vi "Mandelbrot_Top.vi"() -> ()   [LabVIEW 2020]
doc: "This benchmark is designed to demonstrate execution performance improvement when executing FFT and IFFT operations on a GPU."
uses:
  <vilib>/Analysis/1siggen.llb/Ramp Pattern by Delta.vi
  <vilib>/Utility/file.llb/Read Delimited Spreadsheet (DBL).vi
  <vilib>/Ngene/CuLab - GPU Accelerated Toolkit/Toolkit/CuLab.lvlib
  <vilib>/Analysis/NI_AALBase.lvlib
panel:
  out "CuLab Mean Performance Gain":dbl[](array[numeric])=[1.0, 22.05888198839261, 2.294988144455706] format="%#.2g"
  out "Releative Exec Time vs CuLab":cluster{i32[], "all rows":dbl[]}[](graph)=[{[100, 200, 300, 400, 500, 600, 700, 800, 900, 1000], "all rows"=[1.0, 1.0, 1.0, 1.0, 1.0, 1.0, 1.0, 1.0, 1.0, 1.0]}, {[100, 200, 300, 400, 500, 600, 700, 800, 900, 1000], "all rows"=[0.8045912431423006, 2.8737294623342633, 6.2281949138049875, 11.291126277991692, 18.815012396949246, 27.10316550048527, 34.90172708957351, 38.99811295548449, 39.49387679077455, 40.07928325338579]}, {[100, 200, 300, 400, 500, 600, 700, 800, 900, 1000], "all rows"=[2.9876362098895357, 2.6173252742418085, 2.4274383662643, 2.414197215437082, 2.5477456703897334, 2.477240832223878, 2.3481639475839504, 2.0064648536535485, 1.786744893645114, 1.336924181228108]}]
  in  "CuPy CSV":path=path "D:/Ngene/GitHub/culab_examples/Benchmarks/CuPy/results/GeForce_RTX_2080_Ti/Mandelbrot_CuPy.csv"
  out "Execution Time":cluster{i32[], "FFT mean Exec Time":dbl[]}[](graph)=[{[100, 200, 300, 400, 500, 600, 700, 800, 900, 1000], "FFT mean Exec Time"=[0.1258352000004379, 0.13859289999982138, 0.1453709000006711, 0.14599060000000463, 0.1388639000006151, 0.14194279999992432, 0.1489036999992095, 0.17667840000012802, 0.22171379999963392, 0.26985270000022865]}, {[100, 200, 300, 400, 500, 600, 700, 800, 900, 1000], "FFT mean Exec Time"=[0.10124589999941236, 0.398278499999833, 0.9053982999994332, 1.6483982999998261, 2.6127260000002934, 3.8470992000002298, 5.196996300000137, 6.8901241999992635, 8.756337499999972, 10.815502800000104]}, {[100, 200, 300, 400, 500, 600, 700, 800, 900, 1000], "FFT mean Exec Time"=[0.3759498, 0.36274270000000003, 0.3528789, 0.35245010000000004, 0.35378990000000005, 0.3516265, 0.3496503, 0.354499, 0.396146, 0.3607726]}]
  in  "Size Delta":i32=100
  out "GPU Model":string="NVIDIA GeForce RTX 2080 Ti"
  out "CPU Model":string="Intel(R) Core(TM) i7-8700K"
  in  "Max Iterations":i32=1000
  in  "Size Stop":i32=1000
  in  "Size Start":i32=100
  out "Dims H,W":i32[](array[numeric])=[100, 200, 300, 400, 500, 600, 700, 800, 900, 1000] format="%.2p"
  # "Mandelbrot Benchmark"
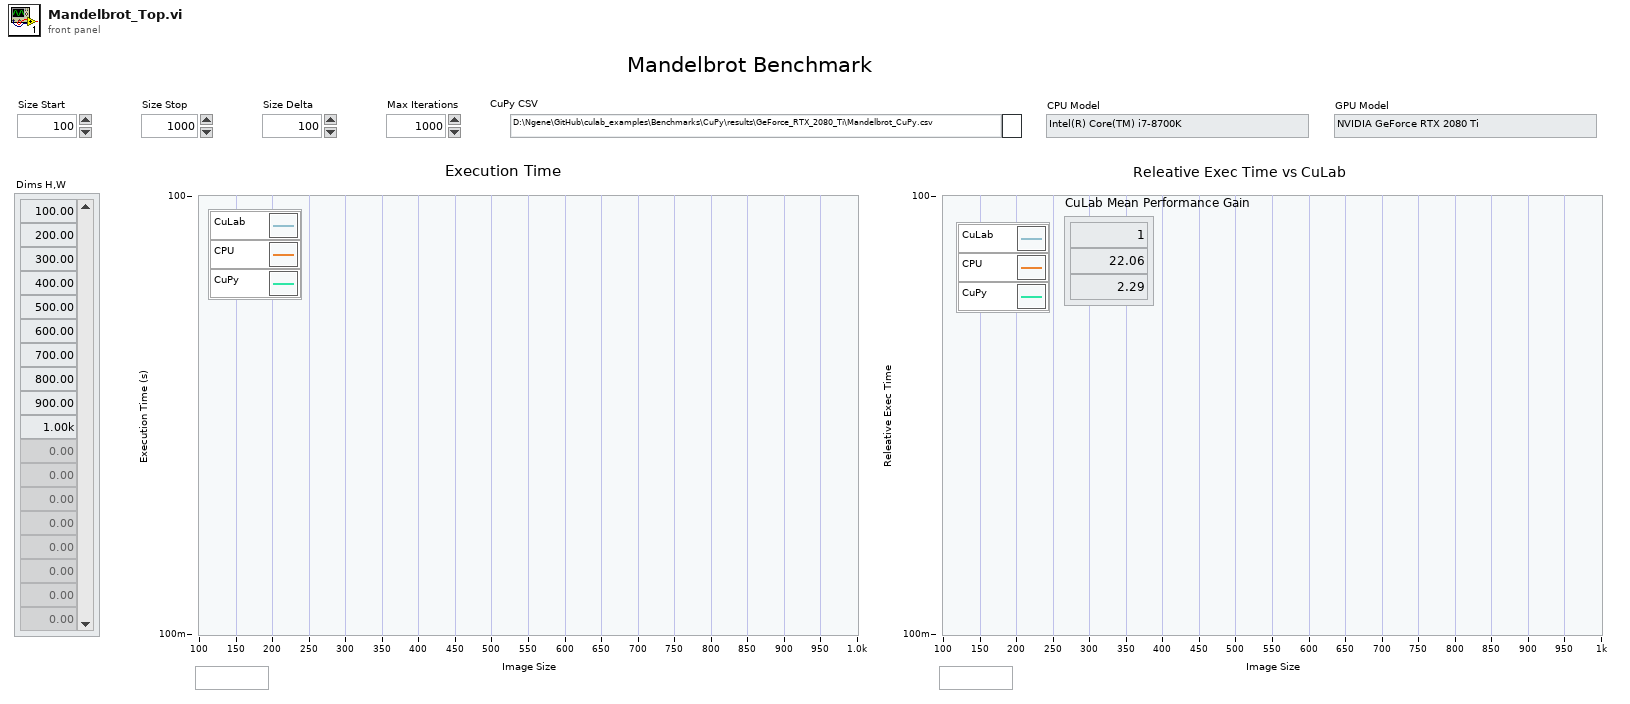
[diagram p1: front panel]
types:
  T1 = typedef "CuLab.lvlib/Properties.ctl" = cluster{"Device ID":i32, "Name":string}
  T2 = typedef "imagedata.ctl" = cluster{"image type":i32, "image depth":i32, "image":u8[], "mask":u8[], "colors":u32[], "Rectangle":cluster{"left":i16, "top":i16, "right":i16, "bottom":i16}}
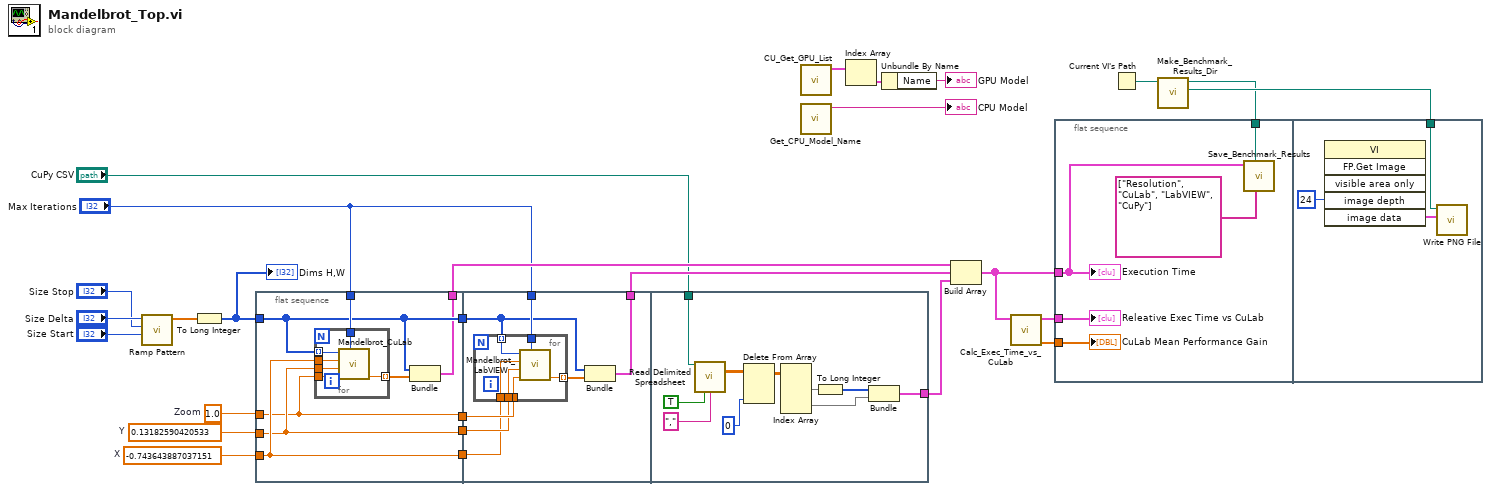
[diagram p0: block diagram]
diagram:
  w15 = 1.0  # Zoom
  w16 = 0.13182590420533  # Y
  w17 = -0.743643887037151  # X
  n1 = call-poly <vilib>:"Ramp Pattern.vi"("start"="Size Start", "end"="Size Stop", "delta"="Size Delta") -> ("Ramp Pattern"=w19:dbl[])  [unwired: 6 in, 2 out]
  n2 = To Long Integer(number=w19) -> (32bit integer=w18:i32[])
  "Dims H,W" <- w18
  n3 = flat-sequence {
    tunnel: [w28] -> w23
    tunnel: [w29] -> w24
    tunnel: w18 -> [w29]
    tunnel: "Max Iterations" -> [w34]
    tunnel: w17 -> [w33]
    tunnel: w16 -> [w32]
    tunnel: w15 -> [w31]
    tunnel: [w33] -> w14
    tunnel: [w32] -> w13
    tunnel: [w31] -> w12
    tunnel: w24 -> [w42]
    tunnel: "Max Iterations" -> [w47]
    tunnel: w14 -> [w44]
    tunnel: w13 -> [w45]
    tunnel: w12 -> [w46]
    tunnel: [w41] -> w10
    tunnel: "CuPy CSV" -> [w63]
    tunnel: [w55] -> w8
    frame #0 {
      n4 = for {
        tunnel: w34 -> [w40]
        tunnel: w33 -> [w39]
        tunnel: w32 -> [w38]
        tunnel: w31 -> [w37]
        tunnel: w29 -> [w35] mode=indexing
        tunnel: [w36] -> w30 mode=indexing
        n5 = call "Mandelbrot_CuLab.vi"("Max_iter"=w40, "Zoom"=w37, "y"=w38, "x"=w39, "Resolution"=w35) -> ("Exec Time"=w36:dbl)  [unwired: 5 in, 1 out]
      }
      n6 = Bundle(w29, w30) -> (w28:cluster{i32[], dbl[]})  [unwired: 1 in]
    }
    frame #1 {
      n7 = for {
        tunnel: w42 -> [w53] mode=indexing
        tunnel: w47 -> [w52]
        tunnel: w46 -> [w51]
        tunnel: w45 -> [w50]
        tunnel: w44 -> [w49]
        tunnel: [w48] -> w43 mode=indexing
        n8 = call "Mandelbrot_LabVIEW.vi"("Max_iter"=w52, "Zoom"=w51, "y"=w50, "x"=w49, "Resolution"=w53) -> ("Exec Time"=w48:dbl)  [unwired: 5 in, 1 out]
      }
      n9 = Bundle(w42, w43) -> (w41:cluster{i32[], dbl[]})  [unwired: 1 in]
    }
    frame #2 {
      n10 = call-poly <vilib>:"Read Delimited Spreadsheet.vi"("file path (dialog if empty)"=w63, "transpose? (F)"=TRUE, "delimiter (\\t)"="," ("delimiter (\\t)")) -> ("all rows"=w61:dbl[][])  [unwired: 7 in, 5 out]
      n11 = Delete From Array(array=w61, index (col)=0 ("disabled index (col)")) -> (array with subset deleted=w59:dbl[][])  [unwired: 2 in, 1 out]
      n12 = Index Array(array=w59) -> (element #1=w58:dbl[], element #2=w56:dbl[])  [unwired: 4 in]
      n13 = To Long Integer(number=w58) -> (32bit integer=w57:i32[])
      n14 = Bundle(w57, "all rows"=w56) -> (w55:cluster{i32[], "all rows":dbl[]})  [unwired: 1 in]
    }
  }
  n15 = call <vilib>:"CU_Get_GPU_List.vi"() -> ("Devices"=w26:T1[])  [unwired: 10 in, 1 out]
  n16 = call "Get_CPU_Model_Name.vi"() -> ("CPU Model"=→"CPU Model":string)  [unwired: 11 in]
  n17 = Index Array(array=w26) -> (element=w25:T1)  [unwired: 1 in]
  n18 = Unbundle By Name(w25) -> ("Name"=→"GPU Model":string)
  n19 = Build Array(w23, w10, w8) -> (w3:cluster{i32[], "all rows":dbl[]}[])
  n20 = call "Calc_Exec_Time_vs_CuLab.vi"("Exec Times"=w3) -> ("Mean Gain"=w1:dbl[], "CuLab Gain"=w2:cluster{"Array":i32[], "all rows":dbl[]}[])  [unwired: 9 in]
  n21 = flat-sequence {
    tunnel: w2 -> [w68]
    tunnel: w1 -> [w67]
    tunnel: w3 -> [w64]
    tunnel: w6 -> [w65]
    tunnel: w7 -> [w70]
    frame #0 {
      n22 = call "Save_Benchmark_Results.vi"("Header"=string[] ["Resolution", "CuLab", "LabVIEW", "CuPy"], "file path (dialog if empty)"=w65, "Execution Time"=w64) -> ()  [unwired: 9 in]
      "Execution Time" <- w64
      "CuLab Mean Performance Gain" <- w67
      "Releative Exec Time vs CuLab" <- w68
    }
    frame #1 {
      n23 = invoke class="VI" method="FP.Get Image"("image depth"=24 ("Image Depth")) -> ("image data"=w71:T2)  [unwired: 5 in, 5 out]
      n24 = call <vilib>:"Write PNG File.vi"("image data"=w71, "path to PNG file"=w70) -> ()  [unwired: 8 in, 2 out]
    }
  }
  n25 = Current VI's Path() -> (path=w4:path)
  n26 = call "Make_Benchmark_Results_Dir.vi"("Caller Path"=w4) -> ("Caller FP Image Path"=w7:path, "CSV_File"=w6:path)  [unwired: 9 in]
